vi "Populate VIs.vi"(8 "error in":errorcluster, 11 "Runner in":refnum<class "Runner.lvclass">) -> (0 "error out":errorcluster, 3 "Runner out":refnum<class "Runner.lvclass">)   [LabVIEW 2026, in "Runner.lvlib" / "Runner.lvclass"]
doc: "Add elements to template based VI."
uses:
  Runner.lvclass
  Runner.lvclass/Runner.ctl
  Interfaces/ILogger/ILogger Messages/Log Msg/Log Msg.lvclass/Log Msg.ctl
  <vilib>/ActorFramework/Message Enqueuer/Message Enqueuer.lvclass/Message Enqueuer.ctl
  Classes/Virtual Instrument/Virtual Instrument.lvclass
  Classes/Virtual Instrument/Virtual Instrument.lvclass/Virtual Instrument.ctl
  Classes/LabVIEW File/LabVIEW File.lvclass/LabVIEW File.ctl
  Classes/Virtual Instrument/Write Python Function Name.vi
  Classes/LabVIEW File/Write Name.vi
  <vilib>/ActorFramework/Message Enqueuer/Enqueue.vi
  Interfaces/ILogger/ILogger Messages/Log Msg/Log Msg.lvclass
  <vilib>/ActorFramework/Message Priority Queue/Priority Enqueue.vi
  Interfaces/ILV File Creator/ILV File Creator.lvclass
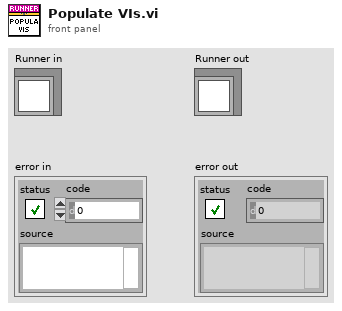
[diagram p1: front panel]
types:
  T1 = typedef "Function--cluster.ctl" = cluster{"name":string, "docstring":string, "input_parameters":T2[], "output_parameters":T2[]}
  T2 = typedef "Parameter--cluster.ctl" = cluster{"name":string, "data_type":string, "container":string, "dimensions":i32, "type_definition":string}
  T3 = typedef "Log Entry--cluster.ctl" = cluster{"Time":timestamp, "Message":string}
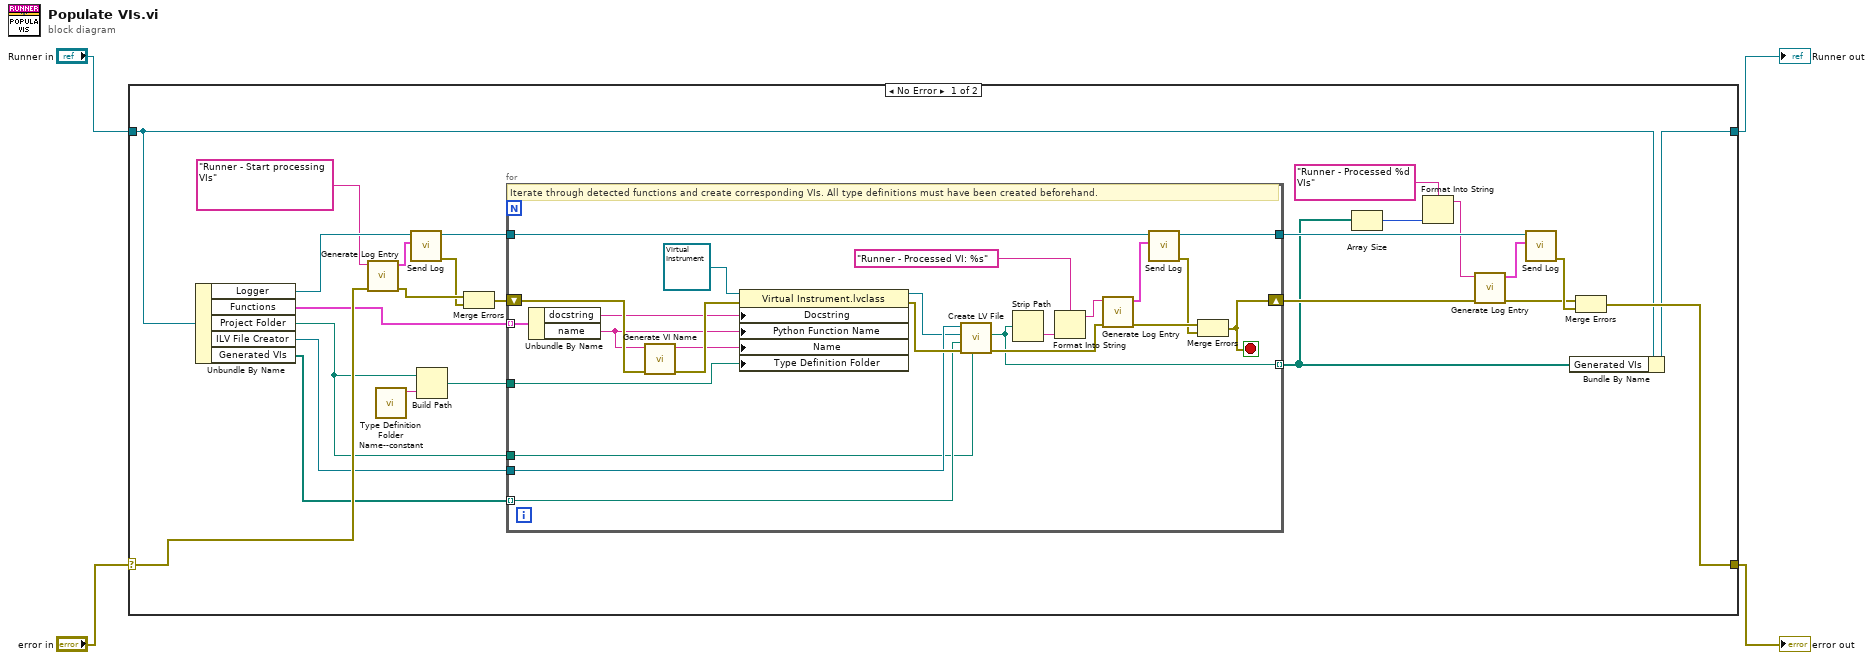
[diagram p0: block diagram]
diagram:
  n1 = case shown="No Error" "error in" {
    selector: "error in" -> [w23 w56]
    tunnel: [w24 w56] -> w3
    tunnel: "Runner in" -> [w8 w55]
    tunnel: [w7 w55] -> w1
    frame No Error {
      n2 = Unbundle By Name(w8) -> ("Logger"=w19:refnum<class "Message Enqueuer.lvclass">, "Functions"=w22:T1[], "Project Folder"=w6:path, "ILV File Creator"=w15:refnum<class "ILV File Creator.lvclass">, "Generated VIs"=w5:path[])
      n3 = call "Generate Log Entry.vi"("error in"=w23, "Message"="Runner - Start processing VIs") -> ("error out"=w30:errorcluster, "Log Entry"=w17:T3)  [unwired: 8 in]
      n4 = call "Type Definition Folder Name--constant.vi"() -> ("Type Definition Folder Name"=w21:string)  [unwired: 11 in]
      n5 = call "Send Log.vi"("Log Entry"=w17, "Message Enqueuer"=w19) -> ("error out"=w28:errorcluster, "Message Enqueuer out"=w18:refnum<class "Message Enqueuer.lvclass">)  [unwired: 8 in]
      n6 = Build Path(base path=w6, name or relative path=w21) -> (appended path=w20:path)
      n7 = Merge Errors(w30, w28) -> (w29:errorcluster)
      n8 = for {
        tunnel: w22 -> [w47] mode=indexing
        tunnel: w20 -> [w31]
        shift-right: [w52] -> w26
        shift-left: w29 -> [w50]
        tunnel: w5 -> [w40] mode=indexing
        tunnel: w18 -> [w46]
        tunnel: [w39] -> w11 mode=indexing
        tunnel: w15 -> [w41]
        tunnel: [w38] -> w13
        tunnel: w6 -> [w32]
        stop <- w52 stop-if-true
        # "Iterate through detected functions and create corresponding VIs. All type definitions must have been created beforehand."
        n9 = Unbundle By Name(w47) -> ("docstring"=w36:string, "name"=w35:string)
        n10 = call "Generate VI Name.vi"("error in"=w50, "Python Function Name"=w35) -> ("error out"=w49:errorcluster, "VI Name"=w37:string)  [unwired: 8 in]
        n11 = property on="Property Node" class="Virtual Instrument.lvclass"(reference=refnum<class "Virtual Instrument.lvclass"> refnum ("Virtual Instrument.lvclass"), error in=w49, "Docstring"=w36, "Python Function Name"=w35, "Name"=w37, "Type Definition Folder"=w31) -> (reference out=w33:refnum<class "Virtual Instrument.lvclass">, error out=w48:errorcluster)
        n12 = call-dynamic "Create LV File.vi"("Output Folder"=w32, "error in"=w48, "Template"=w40, "ILabVIEW File"=w33, "ILV File Creator in"=w41) -> ("error out"=w51:errorcluster, "File Path"=w39:path)  [unwired: 4 in, 1 out]
        n13 = Strip Path(path=w39) -> (name=w42:string)  [unwired: 1 out]
        n14 = Format Into String(format string="Runner - Processed VI: %s", w42) -> (resulting string=w44:string)  [unwired: 2 in, 1 out]
        n15 = call "Generate Log Entry.vi"("error in"=w51, "Message"=w44) -> ("error out"=w54:errorcluster, "Log Entry"=w43:T3)  [unwired: 8 in]
        n16 = call "Send Log.vi"("Log Entry"=w43, "Message Enqueuer"=w46) -> ("error out"=w53:errorcluster, "Message Enqueuer out"=w38:refnum<class "Message Enqueuer.lvclass">)  [unwired: 8 in]
        n17 = Merge Errors(w54, w53) -> (w52:errorcluster)
      }
      n18 = Array Size(array=w11) -> (size(s)=w10:i32)
      n19 = Format Into String(format string="Runner - Processed %d VIs" ("Message"), w10) -> (resulting string=w9:string)  [unwired: 2 in, 1 out]
      n20 = call "Generate Log Entry.vi"("error in"=w26, "Message"=w9) -> ("error out"=w25:errorcluster, "Log Entry"=w14:T3)  [unwired: 8 in]
      n21 = call "Send Log.vi"("Log Entry"=w14, "Message Enqueuer"=w13) -> ("error out"=w27:errorcluster)  [unwired: 8 in, 1 out]
      n22 = Bundle By Name(cluster=w8, "Generated VIs"=w11) -> (w7:refnum<class "Runner.lvclass">)
      n23 = Merge Errors(w25, w27) -> (w24:errorcluster)
    }
    frame Error {
      # "Pass error without actions."
    }
  }
  "error out" <- w3
  "Runner out" <- w1
